vi "Parse XML String for Multiple Nodes.vi"(11 "file (use dialog)":path) -> (3 "Array":string[](array[string]))   [LabVIEW 2025, in "Digital Pattern Sequencer.lvclass"]
doc: "This example demonstrates how to query an XML document by using an XPath expression and returns all the nodes that match the XPath expression."
uses:
  Digital Pattern Sequencer.lvclass
  Digital Pattern Sequencer.lvclass/Digital Pattern Sequencer.ctl
  <resource>/objmgr/DOMUserDefRef.rc
  <vilib>/xml/Load XML String.vi
  <vilib>/xml/NI_XML.lvlib
  <vilib>/xml/XPath/Get All Matched Nodes (String).vi
panel:
  in  "XPath Expression":string="//*[local-name()='FileReference']/@Name"
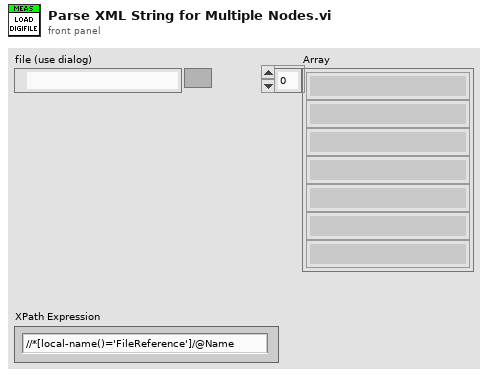
[diagram p1: front panel]
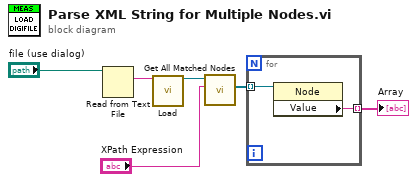
[diagram p0: block diagram]
diagram:
  n1 = Read from Text File(file (use dialog)="file (use dialog)") -> (text=w1:string)  [unwired: 3 in, 3 out]
  n2 = call-poly <vilib>:"Load.vi"("XML string"=w1) -> ("DOM document out"=w4:refnum<k20>)  [unwired: 12 in, 2 out]
  n3 = call-poly <vilib>:"Get All Matched Nodes.vi"("XPath expression"="XPath Expression", "node in"=w4) -> ("node result array"=w6:refnum<k20>[])  [unwired: 7 in, 2 out]
  n4 = for {
    tunnel: w6 -> [w8] mode=indexing
    tunnel: [w7] -> w3 mode=indexing
    n5 = property class="Node"(reference=w8) -> ("Value"=w7:string)  [unwired: 1 in, 2 out]
  }
  "Array" <- w3
